vi "Config_Decode.vi"(8 "error in (no error)":errorcluster={"status"=FALSE, "code"=0, "source"="\"\""}, 11 "Raw package bytes":string) -> (0 "error out":errorcluster={"status"=FALSE, "code"=0, "source"="\"\""}, 2 "status ok":bool, 3 "RigDefinition":string)   [LabVIEW 2026]
doc: "INTENT: Decode versioned configuration. LOGIC: Parse schema version, materialize typed arrays/clusters, reject unknown required fields."
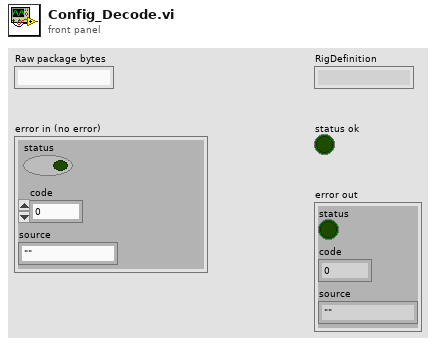
[diagram p1: front panel]
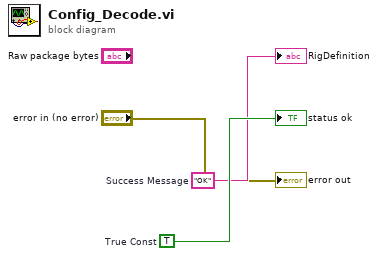
[diagram p0: block diagram]
diagram:
  w3 = TRUE  # True Const
  w2 = "OK"  # Success Message
  "RigDefinition" <- w2
  "status ok" <- w3
  "error out" <- "error in (no error)"
